vi "User Exists.vi"(4 "error in (no error)":errorcluster, 6 "LoginName":string, 7 "EasyUserManager in":refnum<class "EasyUserManager.lvclass">) -> (0 "error out":errorcluster, 2 "User Exists":bool, 3 "EasyUserManager out":refnum<class "EasyUserManager.lvclass">)   [LabVIEW 2024, in "EasyUserManager.lvclass"]
doc: "Check if a user with the provided <B>LoginName</B> exists in the current users file."
uses:
  EasyUserManager.lvclass
  EasyUserManager.lvclass/EasyUserManager.ctl
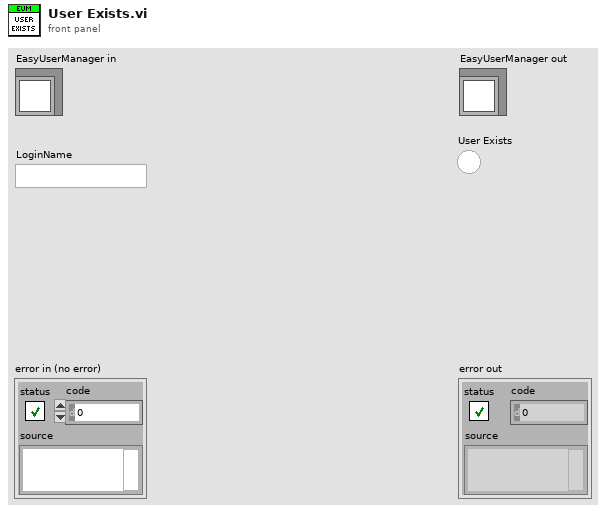
[diagram p1: front panel]
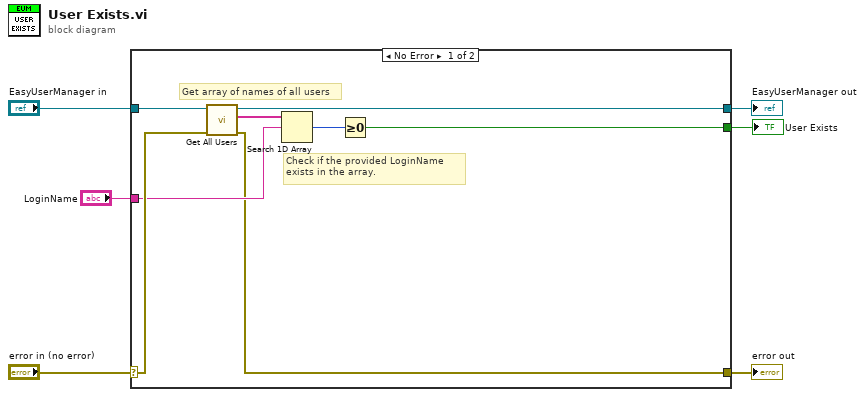
[diagram p0: block diagram]
diagram:
  n1 = case shown="No Error" "error in (no error)" {
    selector: "error in (no error)" -> [w12 w16]
    tunnel: [w7 w16] -> w5
    tunnel: [w14 w15] -> w3
    tunnel: "EasyUserManager in" -> [w13 w15]
    tunnel: "LoginName" -> [w10 _]
    tunnel: [w8 _] -> w1
    frame No Error {
      # "Check if the provided LoginName\nexists in the array."
      # "Get array of names of all users"
      n2 = call "Get All Users.vi"("error in (no error)"=w12, "EasyUserManager in"=w13) -> ("error out"=w7:errorcluster, "Users"=w11:string[], "EasyUserManager out"=w14:refnum<class "EasyUserManager.lvclass">)  [unwired: 3 in]
      n3 = Search 1D Array(1D array=w11, element=w10) -> (index of element=w9:i32)  [unwired: 1 in]
      n4 = Greater Or Equal To 0?(x=w9) -> (x >= 0?=w8:bool)
    }
    frame Error {
      # "Pass error and do nothing."
    }
  }
  "error out" <- w5
  "EasyUserManager out" <- w3
  "User Exists" <- w1
